vi "test_PinMapClient_RegisterPinMapFile_PinMapRegistered.vi"(8 "error in":errorcluster) -> (0 "error out":errorcluster, 2 "result":string, 3 "pass":bool)   [LabVIEW 2021, in "MeasurementServerTests.lvlib" / "Pin Map Tests.lvlib"]
uses:
  Pin Map Tests.lvlib
  gRPC/Generated APIs/ni/measurementlink/pinmap/v1/RPC Messages/ni_measurementlink_pinmap_v1_GetPinMapRequest.ctl
  MeasurementServerTests.lvlib
  Runtime/Clients/Pin Map V1/NI Pin Map V1 Client.lvlib
  gRPC/Generated APIs/ni/measurementlink/pinmap/v1/ni.measurementlink.pinmap.v1.api.lvlib
  Runtime/Clients/Discovery V1/TypeDefs/gRPC Client Cache FGV Action.ctl
  Runtime/Clients/Discovery V1/NI Discovery V1 Client.lvlib
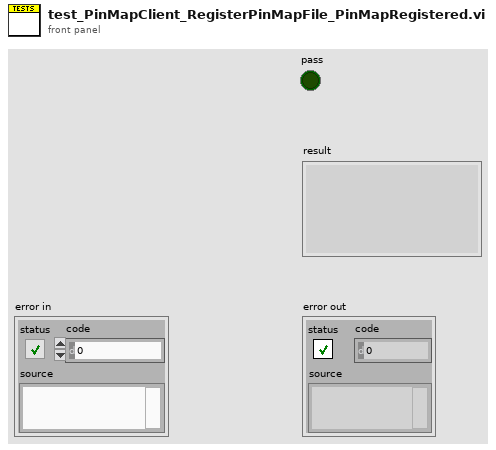
[diagram p1: front panel]
types:
  T1 = typedef "NI Discovery V1 Client.lvlib/gRPC Client Cache FGV Action.ctl" = enum16{"Get Client", "Recreate Client", "Destroy Client", "Update ClusterId"}
  T2 = typedef "ni.measurementlink.pinmap.v1.api.lvlib/ni_measurementlink_pinmap_v1_GetPinMapRequest.ctl" = cluster{"pin_map_id":string}
  T3 = typedef "grpc-lvsupport-release.lvlib/grpcId.ctl" = u64
  T4 = typedef "ni.measurementlink.pinmap.v1.api.lvlib/ni_measurementlink_pinmap_v1_PinMap.ctl" = cluster{"pin_map_id":string}
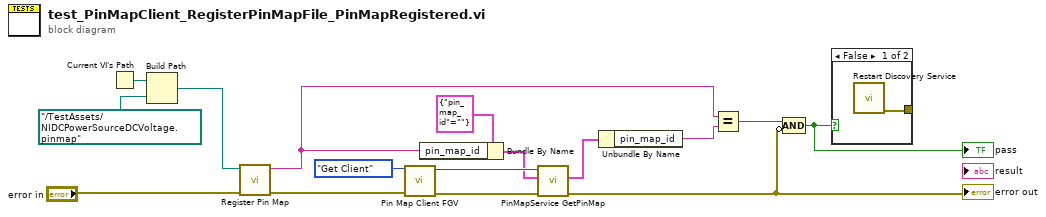
[diagram p0: block diagram]
diagram:
  n1 = Current VI's Path() -> (path=w10:path)
  n2 = Build Path(base path=w10, name or relative path=path "../TestAssets/NIDCPowerSourceDCVoltage.pinmap") -> (appended path=w8:path)
  n3 = call "Register Pin Map.vi"("error in"="error in", "pin map file path"=w8) -> ("error out"=w15:errorcluster, "pin map id"=w2:string)  [unwired: 8 in]
  n4 = call "Pin Map Client FGV.vi"("error in"=w15, "action"=gRPC_Client_Cache_FGV_Action."Get Client") -> ("error out"=w13:errorcluster, "grpc client id"=w14:T3)  [unwired: 7 in, 1 out]
  n5 = Bundle By Name(cluster=T2 {"pin_map_id"=""} ("ni_measurementlink_pinmap_v1_GetPinMapRequest"), "pin_map_id"=w2) -> (w4:T2)
  n6 = call "PinMapService GetPinMap.vi"("error in"=w13, "Request Data"=w4, "gRPC ID"=w14) -> ("error out"=w12:errorcluster, "Response Data"=w11:T4)  [unwired: 6 in, 1 out]
  "error out" <- w12
  n7 = Unbundle By Name(w11) -> ("pin_map_id"=w7:string)
  n8 = Equal?(x=w2, y=w7) -> (x = y?=w6:bool)
  n9 = Compound Arithmetic op=AND(w6, invert w12) -> (w5:bool)
  "pass" <- w5
  n10 = case shown="False" w5 {
    tunnel: [w17 _] -> _
    frame False {
      n11 = call "Restart Discovery Service.vi"() -> ("error out"=w17:errorcluster)  [unwired: 11 in]
    }
    frame True {
    }
  }
